vi "LabVIEW.Main.Read_Test_Status.vi"(8 "error in (no error)":errorcluster caption="Fehler (Eingang, kein Fehler)") -> (0 "error out":errorcluster, 3 "Message_report":string)   [LabVIEW 2019]
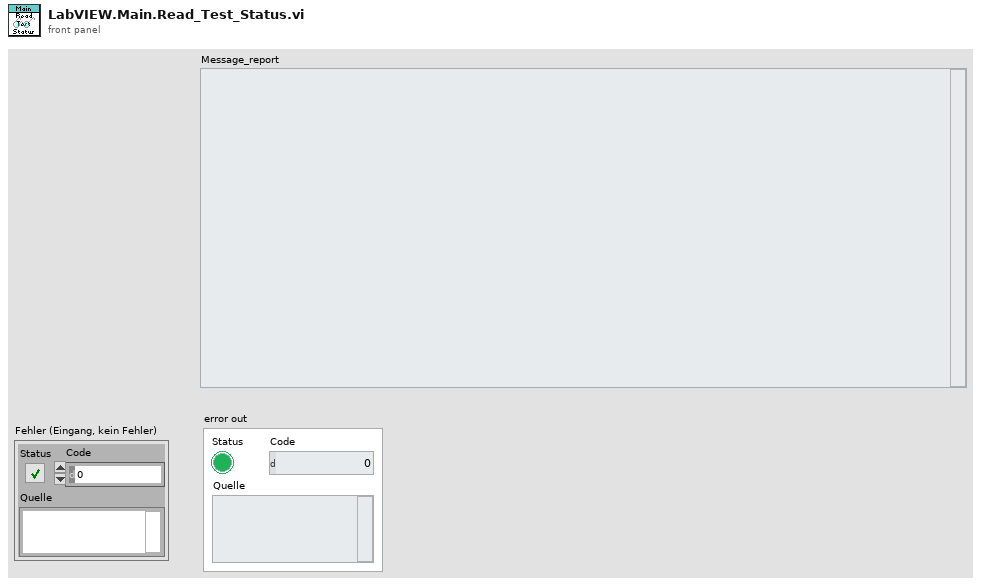
[diagram p1: front panel]
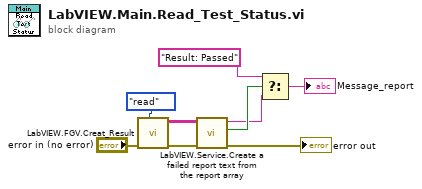
[diagram p0: block diagram]
diagram:
  n1 = call "LabVIEW.FGV.Creat_Result.vi"("Command"=enum16{"write", "read", "clear"}."read", "error in (no error)"="error in (no error)") -> ("error out"=w8:errorcluster, "Angehängtes Array"=w7:string[][])  [unwired: 8 in]
  n2 = call "LabVIEW.Service.Create a failed report text from the report array.vi"("error in (no error)"=w8, "Result[[]]"=w7) -> ("error out"=→"error out":errorcluster, "Passed?"=w4:bool, "report text"=w2:string)  [unwired: 7 in]
  n3 = Select(t="Result: Passed", s=w4, f=w2) -> (s? t:f=→"Message_report":string)
